vi "Connect.vi"   [LabVIEW 2026, in "ORM_API_NetCore.lvlib"]
uses:
  ORM_API_NetCore.lvlib
  <vilib>/Viviota/shared/ORM_DBC_Mssql_netCore.lvlibp/DBC.lvclass
  <vilib>/Viviota/shared/ORM_DBC_MySql_netCore.lvlibp/DBC.lvclass
  <vilib>/Viviota/shared/ORM_DBC_Npgsql_netCore.lvlibp/DBC.lvclass
  <vilib>/Viviota/shared/ORM_DBC_Odbc_netCore.lvlibp/DBC.lvclass
  <vilib>/Viviota/shared/ORM_DBC_Sqlite_netCore.lvlibp/DBC.lvclass
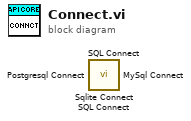
[diagram p0: block diagram]
diagram:
  n1 = call <vilib>:"Sqlite Connect.vi"() -> ()  [unwired: 10 in, 2 out]
  n2 = call <vilib>:"SQL Connect.vi"() -> ()  [unwired: 10 in, 2 out]
  n3 = call <vilib>:"Postgresql Connect.vi"() -> ()  [unwired: 10 in, 2 out]
  n4 = call <vilib>:"MySql Connect.vi"() -> ()  [unwired: 10 in, 2 out]
  n5 = call <vilib>:"SQL Connect.vi"() -> ()  [unwired: 10 in, 2 out]
